vi "configuration UI.vi"() -> ()   [LabVIEW 2015, in "Modbus Module editor node.lvclass"]
doc: "Platypus Framework 1.0.1.65\nNI Systems Engineering - National Instruments"
uses:
  Modbus Module editor node.lvclass
  <vilib>/NI/Configuration Framework/Node/NodeRef.ctl
  <vilib>/NI/Configuration Framework/Node/NISE_CEF_Node.lvclass
  <vilib>/NI/AMC/Message Queue.ctl
  <vilib>/NI/AMC/Message.ctl
  <vilib>/NI/Tools/Keyed Array/KeyedArray.ctl
  <vilib>/NI/Configuration Framework/Node/UserEventRef.ctl
  <vilib>/NI/Configuration Framework/Controls/EventCluster.ctl
  <vilib>/NI/DCAF UI Toolkit/Controls/Configure.ctl
  <vilib>/NI/DCAF UI Toolkit/Controls/Add.ctl
  <vilib>/NI/DCAF UI Toolkit/Controls/Remove.ctl
  <vilib>/NI/DCAF UI Toolkit/Controls/Export.ctl
  module/configuration/modbus class.ctl
  <vilib>/NI/Configuration Framework/Node/NodeChangeEvent.ctl
  <vilib>/NI/DCAF/Tag Editor Core/Table API/Available Tag Menu/channel action event.ctl
  <vilib>/NI/DCAF/Tag Editor Core/Table API/Available Tag Menu/dialog output action.ctl
  <vilib>/NI/Tag Bus Module Framework/channel/TBM channel.lvclass
  <vilib>/NI/Tag Bus/tag/tag descriptor.lvclass
  <vilib>/NI/DCAF/Tag Editor Core/Table API/Table Manager/Call Back Ref Type Def.ctl
  <vilib>/NI/DCAF/Tag Editor Core/Configuration Editor/Classes/Engine Parent/Engine Parent Editor Node.lvclass
  <vilib>/NI/DCAF/Tag Editor Core/Configuration Editor/Classes/Module editor node/module editor node.lvclass
  <vilib>/NI/Configuration Framework/Node/CacheState.ctl
  <vilib>/NI/Configuration Framework/Node/StopEvent.ctl
  <vilib>/NI/Configuration Framework/Node/RefreshUIEvent.ctl
  permissions enum.ctl
  datatypes enum.ctl
  <vilib>/NI/DCAF UI Toolkit/Controls/Import.ctl
  <vilib>/Utility/miscctls.llb/LVRowAndColumnTypeDef.ctl
  <vilib>/NI/DCAF/Tag Editor Core/Table API/Table Manager/references.ctl
  module/configuration/Modbus Module configuration.lvclass
  module/configuration/Modbus Module configuration.lvclass/Modbus Module configuration.ctl
  module/configuration/modbus mapping behavior.ctl
  module/configuration/Read port (502).vi
  module/configuration/Read baud rate.vi
  module/configuration/Read class.vi
  module/configuration/Read flow control (none).vi
  module/configuration/Read parity (even).vi
  module/configuration/Read serial type.vi
  module/configuration/Read unit ID.vi
  module/configuration/Read VISA resource name.vi
  module/configuration/Read IP address.vi
  module/configuration/Read 32-bit first word low.vi
  module/configuration/Read 64-bit first dword low.vi
  module/configuration/Write port (502).vi
  module/configuration/Write baud rate.vi
  module/configuration/Write class.vi
  module/configuration/Write flow control (none).vi
  module/configuration/Write parity (even).vi
  module/configuration/Write serial type.vi
  module/configuration/Write unit ID.vi
  module/configuration/Write VISA resource name.vi
  module/configuration/Write IP address.vi
  module/configuration/Write 32-bit first word low.vi
  module/configuration/Write 64-bit first dword low.vi
  module/configuration/Read modbus channels.vi
  <vilib>/NI/DCAF/Tag Editor Core/Configuration Editor/Classes/Module editor node/Read Module Configuration.vi
  module/configuration/get wire mode.vi
  module/configuration/read force wire mode.vi
  module/configuration/set force wire mode.vi
  module/configuration/set wire mode.vi
  <vilib>/NI/Tag Bus Module Framework/module configuration/TBM module configuration.lvclass
  module/module channel/Modbus Module Channel.lvclass
  <vilib>/NI/DCAF/Tag Editor Core/Table API/Listbox/Multi Column Listbox.lvclass
  <vilib>/NI/Configuration Framework/NISE_CEF_TreeControl.lvlib
  <vilib>/NI/DCAF/Tag Editor Core/Table API/Table Manager.lvlib
  <vilib>/NI/Tools/Keyed Array/Tools_KeyedArray.lvlib
  <vilib>/NI/AMC/AMC.lvlib
  <vilib>/NI/DCAF/Tag Editor Core/Table API/Table Manager/Table Manager.lvclass
  <vilib>/NI/DCAF UI Toolkit/Controls/DCAF UI Elements.lvlib
panel:
  in  "Datatypes Enum":T1
  in  "Permissions Enum":T2
  in  "refresh UI":T3
  in  "stop event":T4
  in  "cache state":T5
  in  "user event out":refnum<user-event>
  in  "node change":T6
  in  "Top Level Tab Control":T7(tab)
  in  "settings":T8
  in  "channel":i32(listbox)=1
  in  "Add Button":T9
  in  "Remove Button":T10
  in  "remap":bool
  in  "64-bit word order":bool
  in  "32-bit word order":bool
  in  "Settings Tab Control":enum32{"TCP", "Serial"}(tab)
  in  "Address":string
  in  "Port (502)":u16=502
  in  "Set Wire Mode?":bool
  in  "Wire Mode":i16(ring) items=["Unknown"=-1, "RS485/Wire4"=0, "RS485/Wire2-EchoDTR"=1, "RS485/Wire2-CtrlDTR"=2, "RS485/Wire2-Auto"=3, "RS232/DTE"=128, "RS232/DCE"=129, "RS232/AUTO"=130]
  in  "Baud Rate":u32
  in  "Flow Control (None)":u16
  in  "Serial Type":enum16{"RTU", "ASCII"}(ring)
  in  "VISA Resource Name":refnum<visa-resource-name>
  in  "Parity":enum16{"None", "Odd", "Even", "Mark", "Space"}(ring)
  in  "Unit ID":u8
  in  "Class":T11
  in  "exportKep":T12
  in  "Import":T13
  in  "Export":T12
  in  "user event":T14
  in  "main queue":T15
  in  "node ref":T16
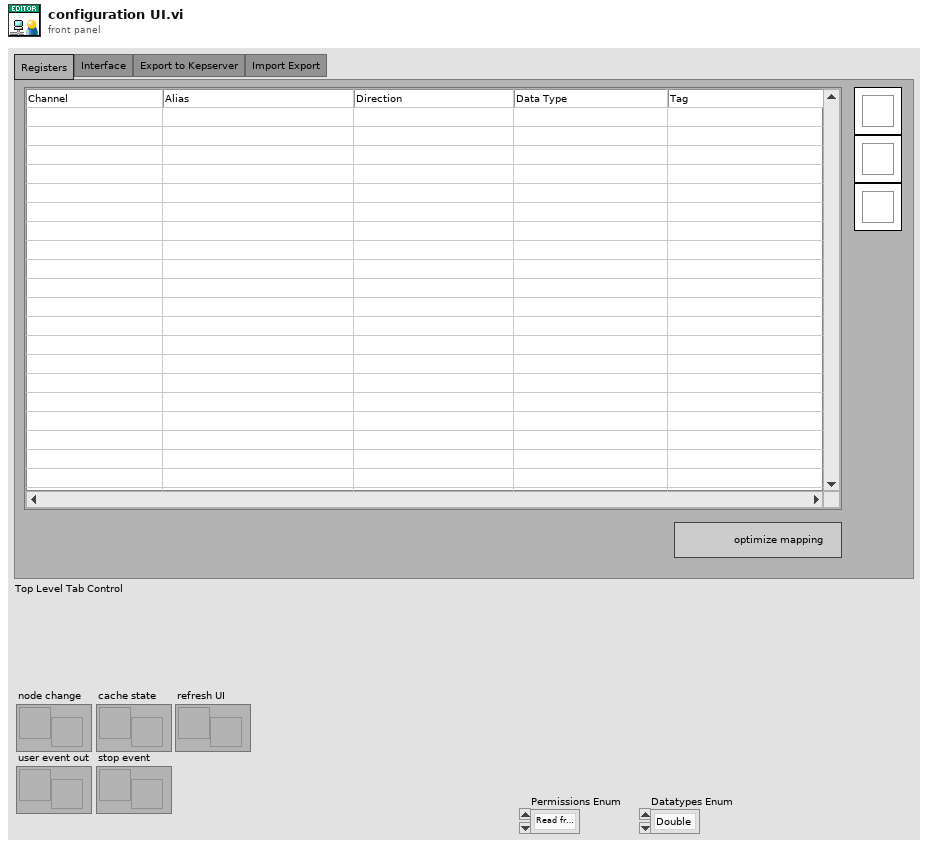
[diagram p1: front panel]
types:
  T1 = typedef "Modbus Module editor node.lvclass/datatypes enum.ctl" = enum16{"Double", "Single", "I64", "I32", "I16", "I8", "U64", "U32", "U16", "U8", "Boolean", "String"}
  T2 = typedef "Modbus Module editor node.lvclass/permissions enum.ctl" = enum16{"Read from MB", "Write to MB"}
  T3 = typedef "NISE_CEF_Node.lvclass/RefreshUIEvent.ctl" = refnum<user-event>
  T4 = typedef "NISE_CEF_Node.lvclass/StopEvent.ctl" = refnum<user-event>
  T5 = typedef "NISE_CEF_Node.lvclass/CacheState.ctl" = refnum<user-event>
  T6 = typedef "NISE_CEF_Node.lvclass/NodeChangeEvent.ctl" = refnum<user-event>
  T7 = enum32{"Registers", "Interface", "Export to Kepserver", "Import Export"}
  T8 = typedef "DCAF UI Elements.lvlib/Configure.ctl" = bool
  T9 = typedef "DCAF UI Elements.lvlib/Add.ctl" = bool
  T10 = typedef "DCAF UI Elements.lvlib/Remove.ctl" = bool
  T11 = typedef "Modbus Module configuration.lvclass/modbus class.ctl" = enum16{"TCP master", "TCP slave", "serial master", "serial slave"}
  T12 = typedef "DCAF UI Elements.lvlib/Export.ctl" = bool
  T13 = typedef "DCAF UI Elements.lvlib/Import.ctl" = bool
  T14 = typedef "NISE_CEF_Node.lvclass/UserEventRef.ctl" = refnum<user-event>
  T15 = typedef "AMC.lvlib/Message Queue.ctl" = refnum<queue>
  T16 = typedef "NISE_CEF_Node.lvclass/NodeRef.ctl" = refnum<data-value>
  T17 = typedef "Table Manager.lvlib/Table Manager.lvclass/references.ctl" = cluster{"stop event":T4, "refresh UI":T3, "cache state":T5, "node change":T6, "user event out":refnum<user-event>, "main queue":T15, "user event":T14}
  T18 = typedef "LVRowAndColumnTypeDef.ctl" = cluster{"Row":i32, "Column":i32}
  T19 = typedef "Table Manager.lvlib/Table Manager.lvclass/object ref.ctl" = cluster{"engine":refnum<data-value>, "Node Ref":refnum<data-value>}
  T20 = typedef "Table Manager.lvlib/Column.lvclass/Column Descriptor.ctl" = cluster{"name":string, "caption":string, "Column Type":T21, "Params":string, "AutoSizeMode":i32, "FillWeight":sgl, "MinWidth":u32, "tooltip":string, "Enum Reference":refnum<vi>, "Channel suffix":string, "Read Only":bool, "Call Back VI":T22, "DT Dependency":i32, "name dependency":i32, "data type":T23, "Custom Column":refnum<class "Column.lvclass">}
  T21 = typedef "Table Manager.lvlib/Column.lvclass/Column Type.ctl" = enum16{"String", "Mapping", "Enum", "Custom"}
  T22 = typedef "Table Manager.lvlib/Table Manager.lvclass/Call Back Ref Type Def.ctl" = refnum<vi>
  T23 = typedef "tag bus.lvlib/tag descriptor.lvclass/Data Type.ctl" = enum16{"Double", "Single", "I64", "I32", "I16", "I8", "U64", "U32", "U16", "U8", "Boolean", "String", "Array of Double", "Array of Single", "Array of I64", "Array of I32", "Array of I16", "Array of I8", "Array of U64", "Array of U32", "Array of U16", "Array of U8", "Array of Boolean", "Array of String"}
  T24 = typedef "Table Manager.lvlib/Table Manager.lvclass/Table Events.ctl" = cluster{"Menu Selection":refnum<user-event>}
  T25 = enum8{"Enabled", "Disabled", "Disabled and Grayed Out"}
  T26 = typedef "Modbus Module configuration.lvclass/modbus mapping behavior.ctl" = enum16{"custom", "optimized"}
  T27 = typedef "Modbus Slave configuration.lvclass/modbus class.ctl" = enum16{"TCP master", "TCP slave", "serial master", "serial slave"}
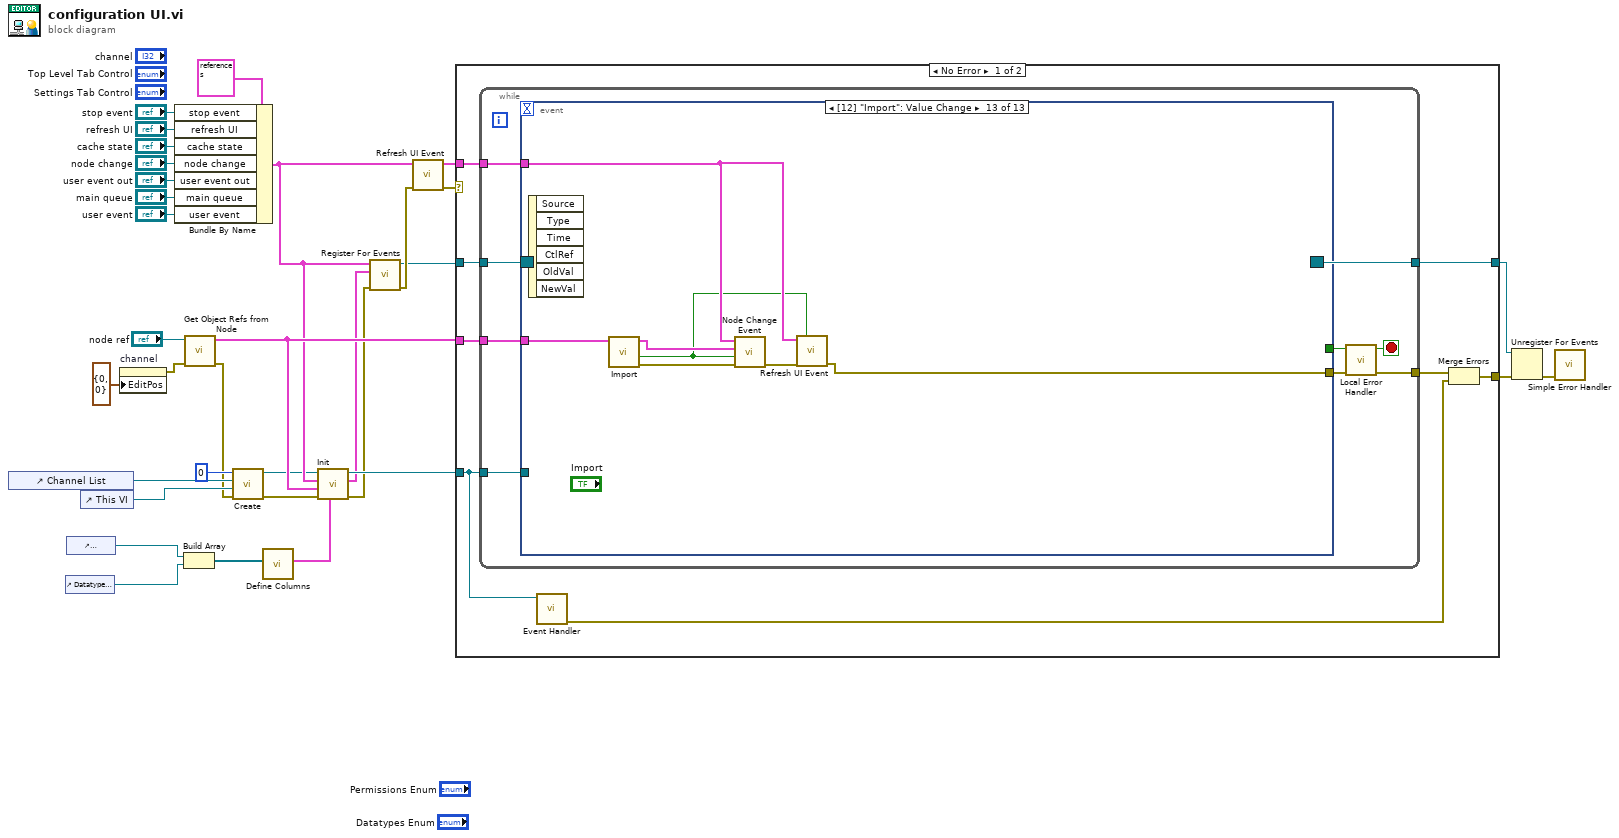
[diagram p0: block diagram]
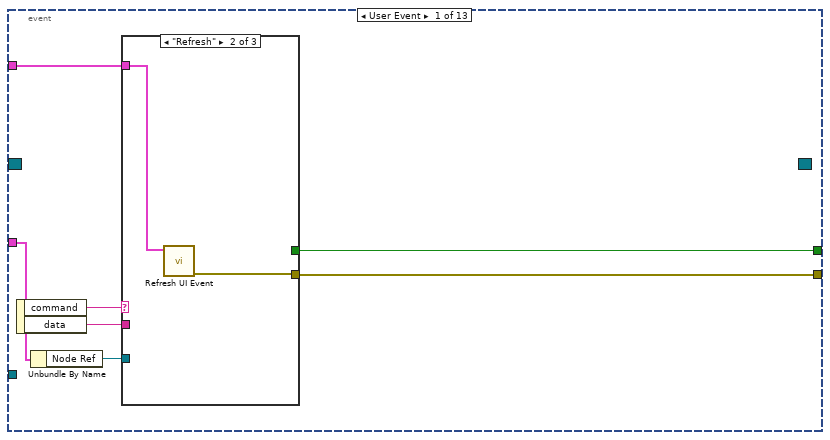
[diagram p2: hidden frame]
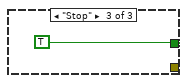
[diagram p4: hidden frame]
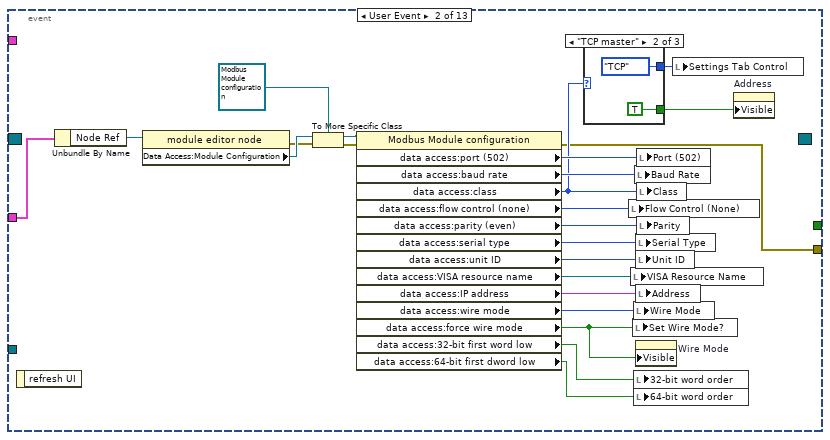
[diagram p5: hidden frame]
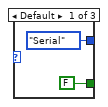
[diagram p6: hidden frame]
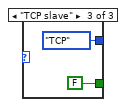
[diagram p7: hidden frame]
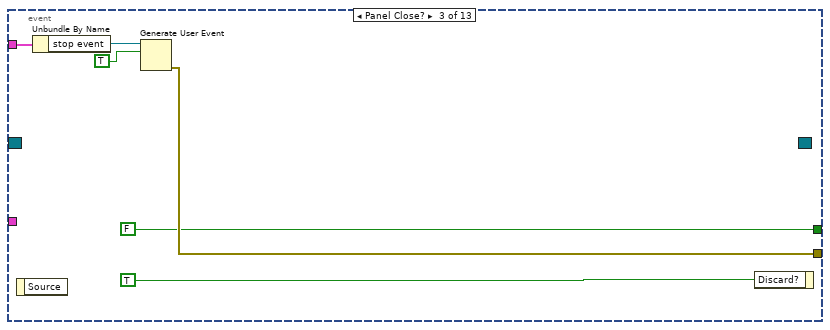
[diagram p8: hidden frame]
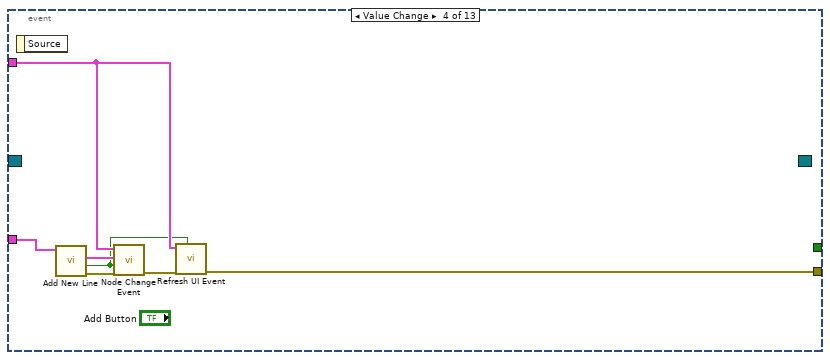
[diagram p9: hidden frame]
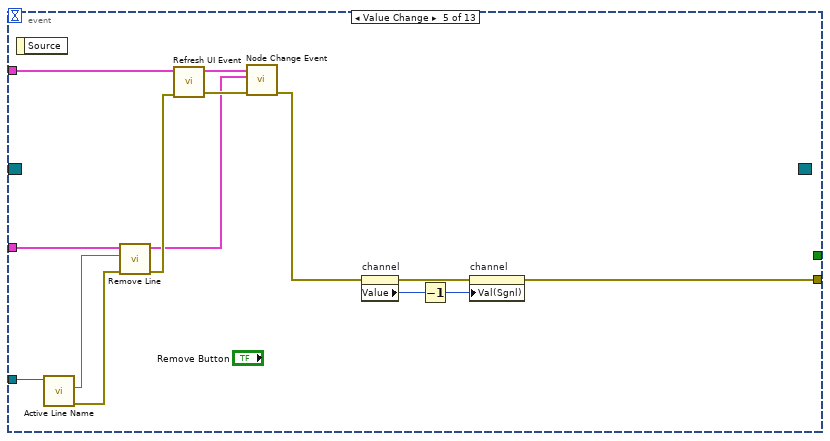
[diagram p10: hidden frame]
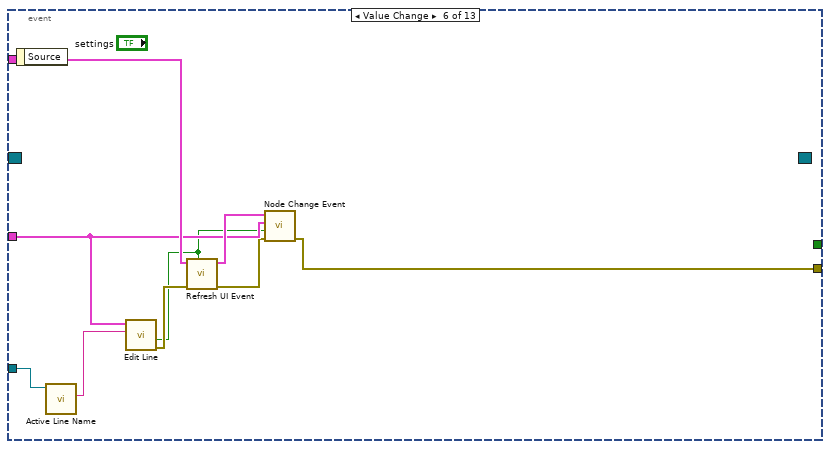
[diagram p11: hidden frame]
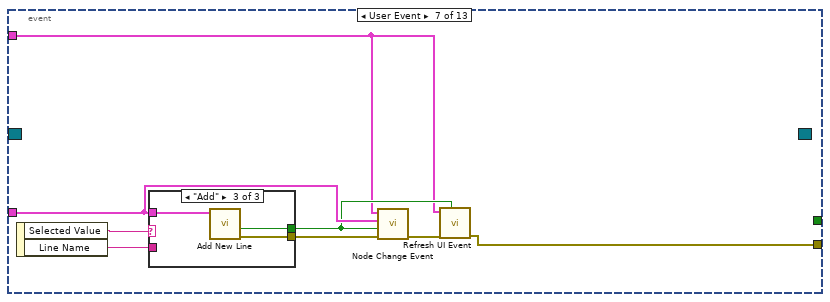
[diagram p12: hidden frame]
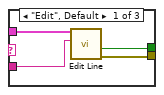
[diagram p13: hidden frame]
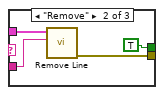
[diagram p14: hidden frame]
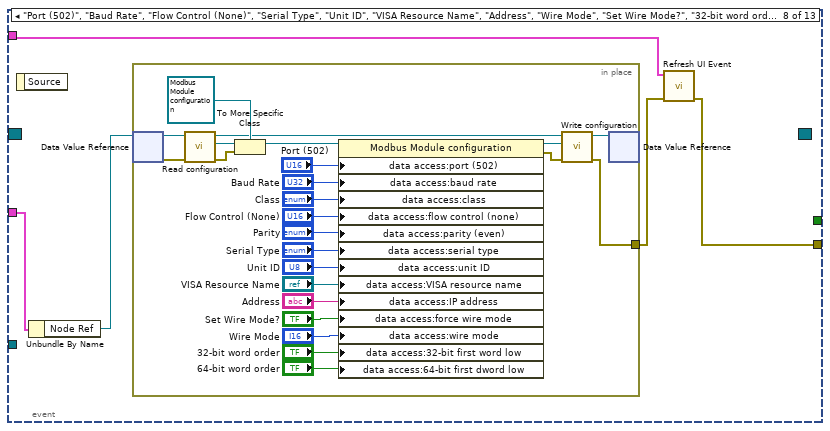
[diagram p15: hidden frame]
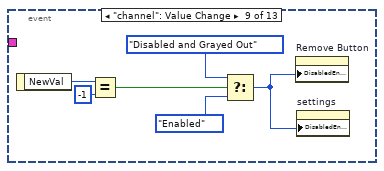
[diagram p16: hidden frame]
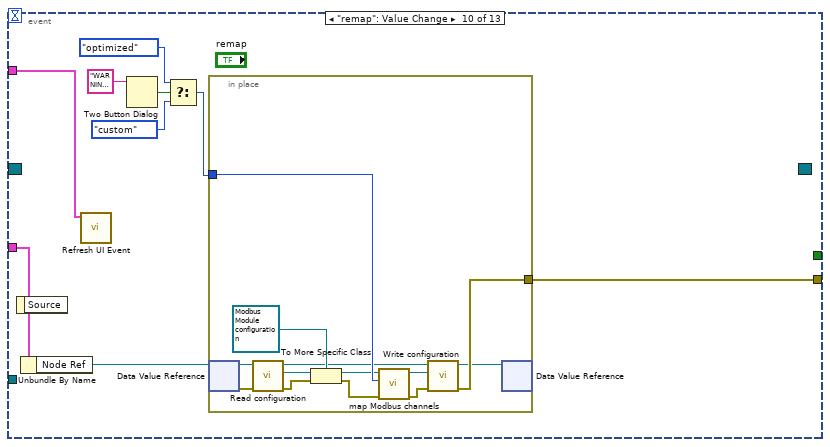
[diagram p17: hidden frame]
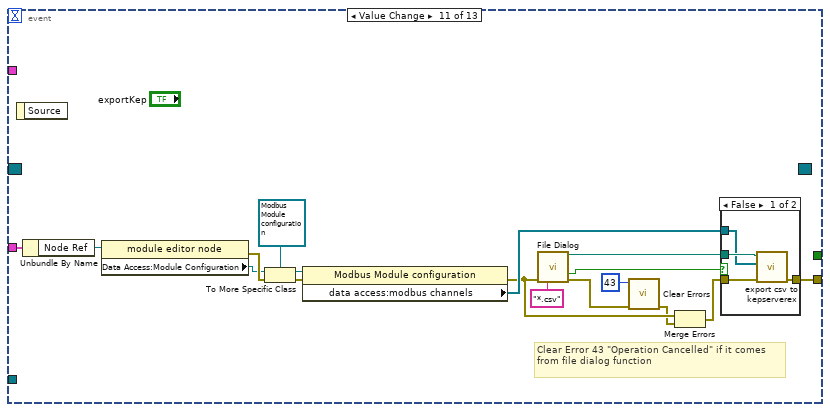
[diagram p18: hidden frame]
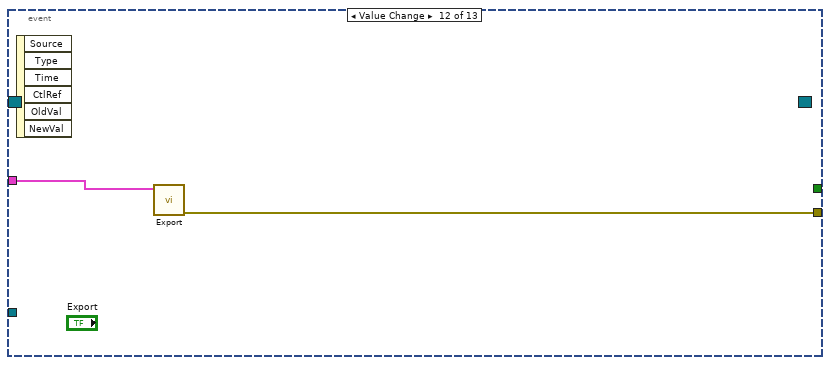
[diagram p20: hidden frame]
diagram:
  n1 = control-ref of="Channel List"() -> (w6:refnum<vi>)
  n2 = control-ref of="Datatypes Enum"() -> (w3:refnum<vi>)
  n3 = control-ref of="Permissions Enum"() -> (w4:refnum<vi>)
  n4 = control-ref of="This VI"() -> (w5:refnum<vi>)
  n5 = property on="channel" class="MCListbox (strict)"("EditPos"=T18 {"Row"=0, "Column"=0} ("Edit Position")) -> (error out=w22:errorcluster)  [unwired: 2 in, 1 out]
  n6 = Bundle By Name(cluster=T17 {"stop event"=refnum, "refresh UI"=refnum, "cache state"=refnum, "node change"=refnum, "user event out"=refnum, "main queue"=refnum, "user event"=refnum} ("References in"), "stop event"="stop event", "refresh UI"="refresh UI", "cache state"="cache state", "node change"="node change", "user event out"="user event out", "main queue"="main queue", "user event"="user event") -> (w13:T17)
  n7 = Build Array(w4, w3) -> (w2:refnum<vi>[])
  n8 = call "Get Object Refs from Node.vi"("error in (no error)"=w22, "Data Value Reference in"="node ref") -> ("error out"=w1:errorcluster, "object Refs"=w15:T19)  [unwired: 8 in]
  n9 = call <vilib>:"Create.vi"("error in (no error)"=w1, "Top VI"=w5, "Listbox"=w6, "Index"=0) -> ("error out"=w8:errorcluster, "reference out"=w9:refnum<class "Multi Column Listbox.lvclass">)  [unwired: 6 in]
  n10 = call "Define Columns.vi"("enum array"=w2) -> ("Column Definitions"=w11:T20[])  [unwired: 10 in]
  n11 = call-dynamic "Init.vi"("Column Descriptors"=w11, "error in (no error)"=w8, "Node object refs"=w15, "Event References"=w13, "Multi Column Listbox in"=w9) -> ("error out"=w12:errorcluster, "Table Events"=w10:T24, "Multi Column Listbox out"=w28:refnum<class "Multi Column Listbox.lvclass">)  [unwired: 4 in]
  n12 = call "Register For Events.vi"("error in (no error)"=w12, "Table Events"=w10, "References in"=w13) -> ("error out"=w25:errorcluster, "Event Registration Refnum"=w24:refnum<event-registration>)  [unwired: 7 in]
  n13 = call "Refresh UI Event.vi"("error in"=w25, "References in"=w13) -> ("error out"=w14:errorcluster, "References out"=w23:T17)  [unwired: 8 in]
  n14 = case shown="No Error" w14 {
    selector: w14 -> [_ w234]
    tunnel: [w41 w233] -> w33
    tunnel: [w34 w234] -> w32
    tunnel: w28 -> [w40 _]
    tunnel: w24 -> [w39 w233]
    tunnel: w23 -> [w38 _]
    tunnel: w15 -> [w37 _]
    frame No Error {
      n15 = while {
        tunnel: [w50] -> w41
        tunnel: [w48] -> w36
        tunnel: w40 -> [w45]
        tunnel: w39 -> [w44]
        tunnel: w38 -> [w43]
        tunnel: w37 -> [w42]
        stop <- w49 stop-if-true
        n16 = event shown="[12] \"Import\": Value Change" {
          selector: w44 -> [_ _ _ _ _ _ _ _ _ _ _ _ _]
          dyn-events: [_ _ _ _ _ _ _ _ _ _ _ _ _] -> w50
          timeout: _ -> [_ _ _ _ _ _ _ _ _ _ _ _ _]
          tunnel: [w57 _ FALSE _ _ _ _ _ _ _ _ _ _] -> w46
          tunnel: [w54 w66 w94 w97 w103 w117 w126 w145 _ w180 w215 w224 w229] -> w47
          tunnel: w45 -> [_ _ _ _ w116 w124 _ _ _ _ _ _ _]
          tunnel: w43 -> [w51 _ w93 w98 w108 w123 w127 w147 _ w183 _ _ w227]
          tunnel: w42 -> [w53 w83 _ w102 w113 w121 w130 w149 _ w182 w208 w225 w232]
          event User Event {
            n17 = event-data() -> ("command"=w56:string, "data"=w55:string)  [unwired: 1 in]
            n18 = Unbundle By Name(w53) -> ("Node Ref"=w52:refnum<data-value>)
            n19 = case shown="\"Refresh\"" w56 {
              tunnel: [_ _ TRUE] -> w57
              tunnel: w55 -> [_ _ _]
              tunnel: [_ w58 _] -> w54
              tunnel: w52 -> [_ _ _]
              tunnel: w51 -> [_ w59 _]
              frame Default {
              }
              frame "Refresh" {
                n20 = call "Refresh UI Event.vi"("References in"=w59) -> ("error out"=w58:errorcluster)  [unwired: 9 in, 1 out]
              }
              frame "Stop" {
              }
            }
          }
          event User Event {
            n21 = event-data() -> ()  [unwired: 1 in, 1 out]
            n22 = Unbundle By Name(w83) -> ("Node Ref"=w82:refnum<data-value>)
            n23 = property class="module editor node"(reference=w82) -> (error out=w68:errorcluster, "Data Access:Module Configuration"=w80:refnum<class "TBM module configuration.lvclass">)  [unwired: 1 in, 1 out]
            n24 = To More Specific Class(target class=refnum<class "Modbus Module configuration.lvclass"> refnum ("tag bus configurable plugin module configuration"), reference=w80, error in=w68) -> (specific class reference=w71:refnum<class "Modbus Module configuration.lvclass">, error out=w67:errorcluster)
            n25 = property class="Modbus Module configuration"(reference=w71, error in=w67) -> (error out=w66:errorcluster, "data access:port (502)"=w75:u16, "data access:baud rate"=w72:u32, "data access:class"=w70:T27, "data access:flow control (none)"=w76:u16, "data access:parity (even)"=w77:u16, "data access:serial type"=w78:enum16{"RTU", "ASCII"}, "data access:unit ID"=w74:u8, "data access:VISA resource name"=w73:refnum<visa-resource-name>, "data access:IP address"=w79:string, "data access:wire mode"=w64:i16, "data access:force wire mode"=w65:bool, "data access:32-bit first word low"=w62:bool, "data access:64-bit first dword low"=w61:bool)  [unwired: 1 out]
            n26 = case shown="\"TCP master\"" w70 {
              tunnel: [enum32{"TCP", "Serial"}."Serial" ("Settings Tab Control") enum32{"TCP", "Serial"}."TCP" ("Settings Tab Control") enum32{"TCP", "Serial"}."TCP" ("Settings Tab Control")] -> w69
              tunnel: [FALSE TRUE FALSE] -> w63
              frame Default {
              }
              frame "TCP master" {
              }
              frame "TCP slave" {
              }
            }
            n27 = local write "Flow Control (None)"(w76) -> ()
            n28 = local write "VISA Resource Name"(w73) -> ()
            n29 = local write "Set Wire Mode?"(w65) -> ()
            n30 = local write "Wire Mode"(w64) -> ()
            n31 = local write "32-bit word order"(w62) -> ()
            n32 = local write "64-bit word order"(w61) -> ()
            n33 = local write "Baud Rate"(w72) -> ()
            n34 = local write "Serial Type"(w78) -> ()
            n35 = local write "Unit ID"(w74) -> ()
            n36 = local write "Address"(w79) -> ()
            n37 = property on="Wire Mode" class="Ring (strict)"("Visible"=w65) -> ()  [unwired: 2 in, 2 out]
            n38 = local write "Port (502)"(w75) -> ()
            n39 = local write "Class"(w70) -> ()
            n40 = local write "Parity"(w77) -> ()
            n41 = local write "Settings Tab Control"(w69) -> ()
            n42 = property on="Address" class="Str"("Visible"=w63) -> ()  [unwired: 2 in, 2 out]
          }
          event Panel Close? {
            n43 = event-data() -> ()  [unwired: 1 in, 1 out]
            n44 = Unbundle By Name(w93) -> ("stop event"=w92:T4)
            n45 = Generate User Event(user event=w92, event data cluster=TRUE ("event data")) -> (error out=w94:errorcluster)  [unwired: 2 in, 1 out]
            n46 = event-data("Discard?"=TRUE) -> ()  [unwired: 1 in, 1 out]
          }
          event Value Change {
            n47 = event-data() -> ()  [unwired: 1 in, 1 out]
            n48 = call "Add New Line.vi"("Object Refs"=w102) -> ("error out"=w100:errorcluster, "Success"=w96:bool, "Object Refs  out"=w101:T19)  [unwired: 8 in]
            n49 = call "Node Change Event.vi"("error in"=w100, "Send"=w96, "object Refs"=w101, "References in"=w98) -> ("error out"=w99:errorcluster)  [unwired: 7 in]
            n50 = call "Refresh UI Event.vi"("Refresh"=w96, "error in"=w99, "References in"=w98) -> ("error out"=w97:errorcluster)  [unwired: 7 in, 1 out]
          }
          event Value Change {
            n51 = event-data() -> ()  [unwired: 1 in, 1 out]
            n52 = call-dynamic "Active Line Name.vi"("Multi Column Listbox in"=w116) -> ("error out"=w114:errorcluster, "Active Line Name"=w115:string)  [unwired: 8 in, 1 out]
            n53 = call "Remove Line.vi"("error in (no error)"=w114, "Active Line Name"=w115, "object Refs in"=w113) -> ("error out"=w110:errorcluster, "object Refs out"=w109:T19)  [unwired: 7 in]
            n54 = call "Refresh UI Event.vi"("error in"=w110, "References in"=w108) -> ("error out"=w111:errorcluster, "References out"=w112:T17)  [unwired: 8 in]
            n55 = call "Node Change Event.vi"("error in"=w111, "object Refs"=w109, "References in"=w112) -> ("error out"=w107:errorcluster)  [unwired: 8 in]
            n56 = property on="channel" class="MCListbox (strict)"(error in=w107) -> (error out=w104:errorcluster, "Value"=w106:i32)  [unwired: 1 in, 1 out]
            n57 = Decrement(x=w106) -> (x-1=w105:i32)
            n58 = property on="channel" class="MCListbox (strict)"(error in=w104, "Val(Sgnl)"=w105) -> (error out=w103:errorcluster)  [unwired: 1 in, 1 out]
          }
          event Value Change {
            n59 = event-data() -> ()  [unwired: 1 in, 1 out]
            n60 = call-dynamic "Active Line Name.vi"("Multi Column Listbox in"=w124) -> ("Active Line Name"=w125:string)  [unwired: 8 in, 2 out]
            n61 = call "Edit Line.vi"("Line Name"=w125, "object Refs"=w121) -> ("error out"=w120:errorcluster, "Change"=w118:bool)  [unwired: 8 in]
            n62 = call "Refresh UI Event.vi"("Refresh"=w118, "error in"=w120, "References in"=w123) -> ("error out"=w119:errorcluster, "References out"=w122:T17)  [unwired: 7 in]
            n63 = call "Node Change Event.vi"("error in"=w119, "Send"=w118, "object Refs"=w121, "References in"=w122) -> ("error out"=w117:errorcluster)  [unwired: 7 in]
          }
          event User Event {
            n64 = event-data() -> ("Selected Value"=w133:string, "Line Name"=w132:string)  [unwired: 1 in]
            n65 = case shown="\"Add\"" w133 {
              tunnel: w132 -> [w136 w140 _]
              tunnel: w130 -> [w137 w141 w144]
              tunnel: [w134 TRUE ("Success") w143] -> w128
              tunnel: [w135 w139 w142] -> w129
              frame "Edit", Default {
                n66 = call "Edit Line.vi"("Line Name"=w136, "object Refs"=w137) -> ("error out"=w135:errorcluster, "Change"=w134:bool)  [unwired: 8 in]
              }
              frame "Remove" {
                n67 = call "Remove Line.vi"("Active Line Name"=w140, "object Refs in"=w141) -> ("error out"=w139:errorcluster)  [unwired: 8 in, 1 out]
              }
              frame "Add" {
                n68 = call "Add New Line.vi"("Object Refs"=w144) -> ("error out"=w142:errorcluster, "Success"=w143:bool)  [unwired: 8 in, 1 out]
              }
            }
            n69 = call "Node Change Event.vi"("error in"=w129, "Send"=w128, "object Refs"=w130, "References in"=w127) -> ("error out"=w131:errorcluster)  [unwired: 7 in]
            n70 = call "Refresh UI Event.vi"("Refresh"=w128, "error in"=w131, "References in"=w127) -> ("error out"=w126:errorcluster)  [unwired: 7 in, 1 out]
          }
          event "Port (502)", "Baud Rate", "Flow Control (None)", "Serial Type", "Unit ID", "VISA Resource Name", "Address", "Wire Mode", "Set Wire Mode?", "32-bit word order", "64-bit word order", "Parity": Value Change {
            n71 = event-data() -> ()  [unwired: 1 in, 1 out]
            n72 = Unbundle By Name(w149) -> ("Node Ref"=w148:refnum<data-value>)
            n73 = in-place {
              in-place-border: [w155] -> w146
              n74 = in-place-dvr #1(w148) -> (w163:refnum<class "module editor node.lvclass">, w153:errorcluster)
              n75 = call-dynamic "Read configuration.vi"("error in"=w153, "NISE_CEF_serializable node in"=w163) -> ("error out"=w154:errorcluster, "configuration"=w161:refnum<class "NISE_CEF_serializable configuration.lvclass">, "NISE_CEF_serializable node out"=w159:refnum<class "module editor node.lvclass">)  [unwired: 7 in]
              n76 = To More Specific Class(target class=refnum<class "Modbus Module configuration.lvclass"> refnum ("Modbus Module configuration"), reference=w161, error in=w154) -> (specific class reference=w160:refnum<class "Modbus Module configuration.lvclass">)  [unwired: 1 out]
              n77 = property class="Modbus Module configuration"(reference=w160, "data access:port (502)"="Port (502)", "data access:baud rate"="Baud Rate", "data access:class"="Class", "data access:flow control (none)"="Flow Control (None)", "data access:parity (even)"="Parity", "data access:serial type"="Serial Type", "data access:unit ID"="Unit ID", "data access:VISA resource name"="VISA Resource Name", "data access:IP address"="Address", "data access:force wire mode"="Set Wire Mode?", "data access:wire mode"="Wire Mode", "data access:32-bit first word low"="32-bit word order", "data access:64-bit first dword low"="64-bit word order") -> (reference out=w158:refnum<class "Modbus Module configuration.lvclass">, error out=w156:errorcluster)  [unwired: 1 in]
              n78 = call-dynamic "Write configuration.vi"("error in"=w156, "configuration"=w158, "NISE_CEF_serializable node in"=w159) -> ("error out"=w155:errorcluster, "NISE_CEF_serializable node out"=w157:refnum<class "module editor node.lvclass">)  [unwired: 7 in]
              n79 = in-place-dvr #1(w157) -> ()  [unwired: 2 out]
            }
            n80 = call "Refresh UI Event.vi"("error in"=w146, "References in"=w147) -> ("error out"=w145:errorcluster)  [unwired: 8 in, 1 out]
          }
          event "channel": Value Change {
            n81 = event-data() -> ("NewVal"=w179:i32)  [unwired: 1 in]
            n82 = Equal?(x=w179, y=-1) -> (x = y?=w176:bool)
            n83 = Select(t=T25."Disabled and Grayed Out" ("Disabled"), s=w176, f=T25."Enabled" ("Disabled")) -> (s? t:f=w174:T25)
            n84 = property on="Remove Button" class="Bool"("DisabledEnum"=w174) -> ()  [unwired: 2 in, 2 out]
            n85 = property on="settings" class="Bool"("DisabledEnum"=w174) -> ()  [unwired: 2 in, 2 out]
          }
          event "remap": Value Change {
            n86 = event-data() -> ()  [unwired: 1 in, 1 out]
            n87 = Unbundle By Name(w182) -> ("Node Ref"=w181:refnum<data-value>)
            n88 = call "Refresh UI Event.vi"("References in"=w183) -> ()  [unwired: 9 in, 2 out]
            n89 = Two Button Dialog(message="WARNING! This will reorder register mappings and cannot be undone. Press \"OK\" to proceed or \"Cancel\" to keep current mappings.") -> (T button?=w187:bool)  [unwired: 2 in]
            n90 = Select(t=modbus_mapping_behavior."optimized" ("Mapping"), s=w187, f=modbus_mapping_behavior."custom" ("Mapping")) -> (s? t:f=w184:T26)
            n91 = in-place {
              in-place-border: w184 -> [w201]
              in-place-border: [w193] -> w180
              n92 = in-place-dvr #2(w181) -> (w200:refnum<class "module editor node.lvclass">, w199:errorcluster)
              n93 = call-dynamic "Read configuration.vi"("error in"=w199, "NISE_CEF_serializable node in"=w200) -> ("error out"=w195:errorcluster, "configuration"=w191:refnum<class "NISE_CEF_serializable configuration.lvclass">, "NISE_CEF_serializable node out"=w189:refnum<class "module editor node.lvclass">)  [unwired: 7 in]
              n94 = To More Specific Class(target class=refnum<class "Modbus Module configuration.lvclass"> refnum ("Modbus Slave configuration in"), reference=w191, error in=w195) -> (specific class reference=w197:refnum<class "Modbus Module configuration.lvclass">, error out=w196:errorcluster)
              n95 = call "map Modbus channels.vi"("error in"=w196, "mapping"=w201, "Modbus Slave configuration in"=w197) -> ("error out"=w194:errorcluster, "Modbus Slave configuration out"=w190:refnum<class "Modbus Module configuration.lvclass">)  [unwired: 7 in]
              n96 = call-dynamic "Write configuration.vi"("error in"=w194, "configuration"=w190, "NISE_CEF_serializable node in"=w189) -> ("error out"=w193:errorcluster, "NISE_CEF_serializable node out"=w192:refnum<class "module editor node.lvclass">)  [unwired: 7 in]
              n97 = in-place-dvr #2(w192) -> ()  [unwired: 2 out]
            }
          }
          event Value Change {
            # "Clear Error 43 \"Operation Cancelled\" if it comes from file dialog function"
            n98 = event-data() -> ()  [unwired: 1 in, 1 out]
            n99 = Unbundle By Name(w208) -> ("Node Ref"=w207:refnum<data-value>)
            n100 = property class="module editor node"(reference=w207) -> (error out=w214:errorcluster, "Data Access:Module Configuration"=w212:refnum<class "TBM module configuration.lvclass">)  [unwired: 1 in, 1 out]
            n101 = To More Specific Class(target class=refnum<class "Modbus Module configuration.lvclass"> refnum ("tag bus configurable plugin module configuration"), reference=w212, error in=w214) -> (specific class reference=w211:refnum<class "Modbus Module configuration.lvclass">, error out=w213:errorcluster)
            n102 = property class="Modbus Module configuration"(reference=w211, error in=w213) -> (error out=w203:errorcluster, "data access:modbus channels"=w209:refnum<class "Modbus Module Channel.lvclass">[])  [unwired: 1 out]
            n103 = call "File Dialog"("error in"=w203, "pattern (all files)"="*.csv") -> ("selected path"=w218:path, "cancelled"=w216:bool, "error out"=w206:errorcluster)  [unwired: 10 in, 1 out]
            n104 = call <vilib>:"Clear Errors.vi"("error in (no error)"=w206, "specific error code to clear (0: all)"=43) -> ("error out"=w202:errorcluster)  [unwired: 4 in, 1 out]
            n105 = Merge Errors(w203, w202) -> (w204:errorcluster)
            n106 = case shown="False" w216 {
              tunnel: w218 -> [w220 _]
              tunnel: w204 -> [w221 w223]
              tunnel: [w222 w223] -> w215
              tunnel: w209 -> [w219 _]
              frame False {
                n107 = call "export csv to kepserverex.vi"("error in"=w221, "modbus channels"=w219, "selected path"=w220) -> ("error out"=w222:errorcluster)  [unwired: 8 in]
              }
              frame True {
              }
            }
          }
          event Value Change {
            n108 = event-data() -> ()  [unwired: 1 in, 6 out]
            n109 = call "Export.vi"("Objects"=w225) -> ("error out"=w224:errorcluster)  [unwired: 10 in]
          }
          event Value Change {
            n110 = event-data() -> ()  [unwired: 1 in, 6 out]
            n111 = call "Import.vi"("Objects in"=w232) -> ("error out"=w230:errorcluster, "Update"=w226:bool, "Objects out"=w228:T19)  [unwired: 8 in]
            n112 = call "Node Change Event.vi"("error in"=w230, "Send"=w226, "object Refs"=w228, "References in"=w227) -> ("error out"=w231:errorcluster)  [unwired: 7 in]
            n113 = call "Refresh UI Event.vi"("Refresh"=w226, "error in"=w231, "References in"=w227) -> ("error out"=w229:errorcluster)  [unwired: 7 in, 1 out]
          }
        }
        n114 = call "Local Error Handler.vi"("error in (no error)"=w47, "Boolean in"=w46) -> ("error out"=w48:errorcluster, "Boolean out"=w49:bool)  [unwired: 8 in]
      }
      n115 = call-dynamic "Event Handler.vi"("Listbox in"=w40) -> ("error out"=w35:errorcluster)  [unwired: 9 in, 1 out]
      n116 = Merge Errors(w36, w35) -> (w34:errorcluster)
    }
    frame Error {
    }
  }
  n117 = Unregister For Events(event registration refnum=w33, error in=w32) -> (error out=w30:errorcluster)
  n118 = call <vilib>:"Simple Error Handler.vi"("error in (no error)"=w30) -> ()  [unwired: 4 in, 5 out]
